vi "SP - get value.vi"(8 "error in (no error)":errorcluster, 11 "JSON string":string) -> (0 "error out":errorcluster, 3 "value":string)   [LabVIEW 2020, in "ui-testing.lvlib"]
doc: "copyright: Thomas Zilliox©"
uses:
  ui-testing.lvlib
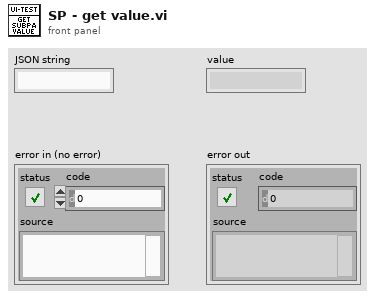
[diagram p1: front panel]
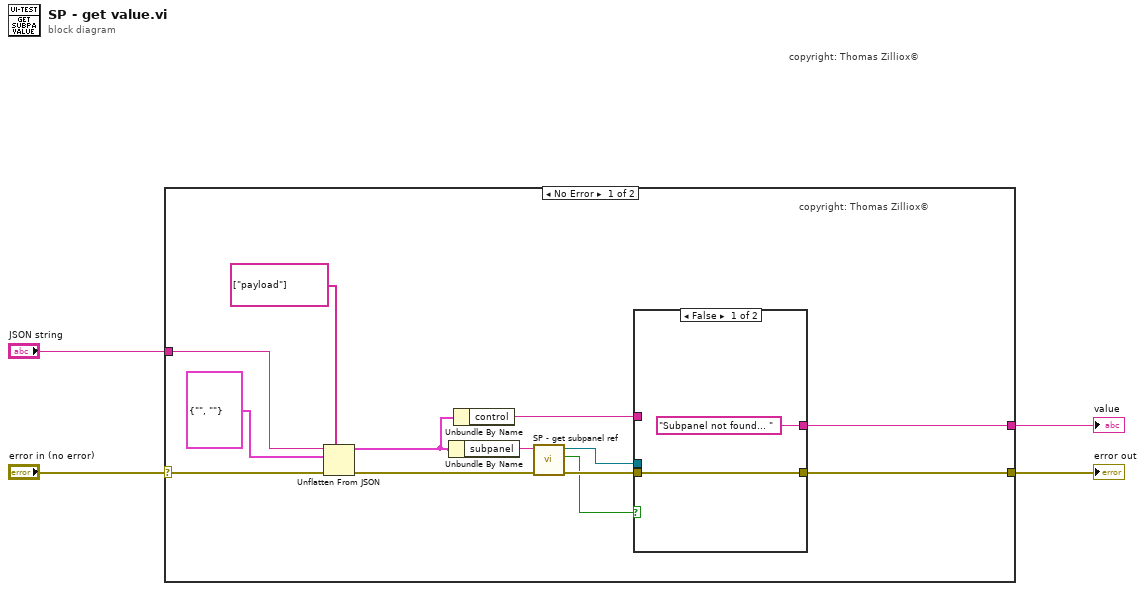
[diagram p0: block diagram]
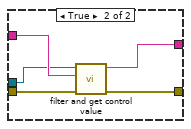
[diagram p2: hidden frame]
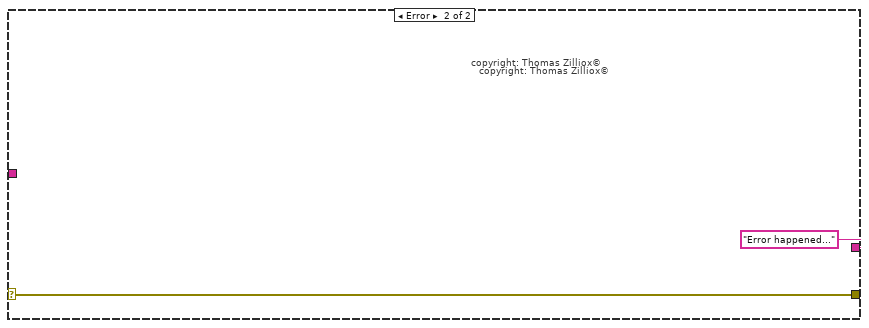
[diagram p3: hidden frame]
diagram:
  # "copyright: Thomas Zilliox©"
  n1 = case shown="No Error" "error in (no error)" {
    selector: "error in (no error)" -> [w13 w26]
    tunnel: "JSON string" -> [w15 _]
    tunnel: [w14 w26] -> w3
    tunnel: [w10 "Error happened..."] -> w1
    frame No Error {
      # "copyright: Thomas Zilliox©"
      n2 = Unflatten From JSON(path=string[] ["payload"], JSON string=w15, type and defaults=cluster{"subpanel":string, "control":string} {"subpanel"="", "control"=""}, error in (no error)=w13) -> (value=w11:cluster{"subpanel":string, "control":string}, error out=w16:errorcluster)  [unwired: 3 in]
      n3 = Unbundle By Name(w11) -> ("subpanel"=w9:string)
      n4 = Unbundle By Name(w11) -> ("control"=w5:string)
      n5 = call "SP - get subpanel ref.vi"("error in (no error)"=w16, "subpanel"=w9) -> ("error out"=w8:errorcluster, "subpanel found ?"=w6:bool, "subpanel VI ref"=w7:refnum<vi>)  [unwired: 6 in, 1 out]
      n6 = case shown="False" w6 {
        tunnel: [w19 w21] -> w14
        tunnel: w7 -> [_ w23]
        tunnel: w8 -> [w19 w20]
        tunnel: ["Subpanel not found... " ("result string") w22] -> w10
        tunnel: w5 -> [_ w24]
        frame False {
        }
        frame True {
          n7 = call "filter and get control value.vi"("error in (no error)"=w20, "Control label"=w24, "VI (Caller)"=w23) -> ("error out"=w21:errorcluster, "Value"=w22:string)  [unwired: 7 in]
        }
      }
    }
    frame Error {
      # "copyright: Thomas Zilliox©"
      # "copyright: Thomas Zilliox©"
    }
  }
  "error out" <- w3
  "value" <- w1
